vi "from string.vi"(8 "error in":errorcluster, 9 "data":string, 10 "version":string, 11 "CEF_Configuration in":refnum<class "XY Plotter configuration.lvclass">) -> (0 "error out":errorcluster, 3 "CEF_Configuration out":refnum<class "XY Plotter configuration.lvclass">)   [LabVIEW 2025, in "XY Plotter.lvlib" / "XY Plotter configuration.lvclass"]
doc: "Provides an interface for loading a module configuration from a file or other serialized data source. It is recommended that all children of this class store data in two sets--data required for its own initialization, and any data required for parent initialization--and that each implementation uses the <b>Call Parent Method</b> primitive to de-serialize parent information.Copyright 2017 National Instruments Corporation\n\nLicensed under the Apache License, Version 2.0 (the \"License\"); you may not use this file except in compliance with the License. You may obtain a copy of the License at http://www.apache.org/licenses/LICENSE-2.0\nUnless required by applicable law or agreed to in writing, software distributed under the License is distributed on an \"AS IS\" BASIS, WITHOUT WARRANTIES OR CONDITIONS OF ANY KIND, either express or implied. See the License for the specific language governing permissions and limitations under the License."
uses:
  XY Plotter configuration.lvclass
  XY Plotter.ctl
  XY Plotter configuration.lvclass/XY Plotter configuration.ctl
  4cdf8148-81d7-474d-a8fa-f40dbeba2f75.vi
  <vilib>/JDP Science/JSONtext/JSON text to Variant.vi
  <vilib>/JDP Science/JSONtext/LVClass Serializer/JSONtext LVClass Serializer.lvclass
  Users/Public/Documents/Sandia National Labs/TSS Plugin/CEF.lvlibp/serializable configuration/CEF_serializable configuration.lvclass
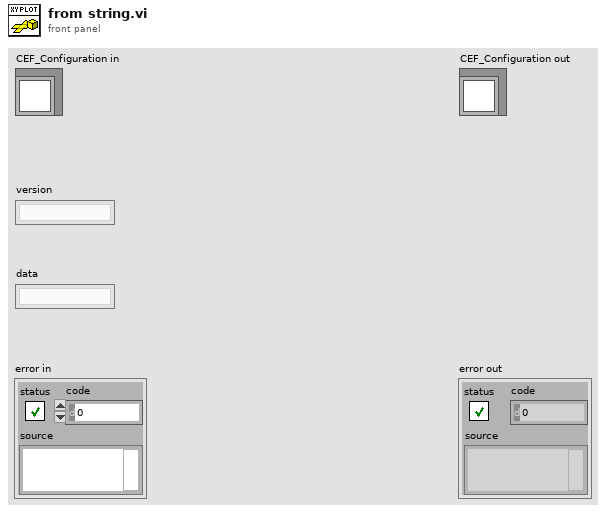
[diagram p1: front panel]
types:
  T1 = typedef "XY Plotter.lvlib/XY Plotter configuration.lvclass/XY Plotter.ctl" = cluster{"Data Rate":i32, "Y-Scales":cluster{"Label":string, "Max":dbl, "Min":dbl, "Unit":enum16{"---", "V", "mA", "sec", "dB", "deg", "in/s", "in", "lbf", "Hz", "psi", "gpm"}, "Visible":bool}[], "Note":string, "History Length":i32, "DataLog Path":path, "Plot type":bool, "X-Scales":cluster{"Label":string, "Max":dbl, "Min":dbl, "Unit":enum16{"---", "V", "mA", "sec", "dB", "deg", "in/s", "in", "lbf", "Hz", "psi", "gpm"}, "Visible":bool}[], "Plot List":cluster{"Plot Name":string, "X Scale Index":u32, "Y Scale Index":u32, "Visible":bool}[]}
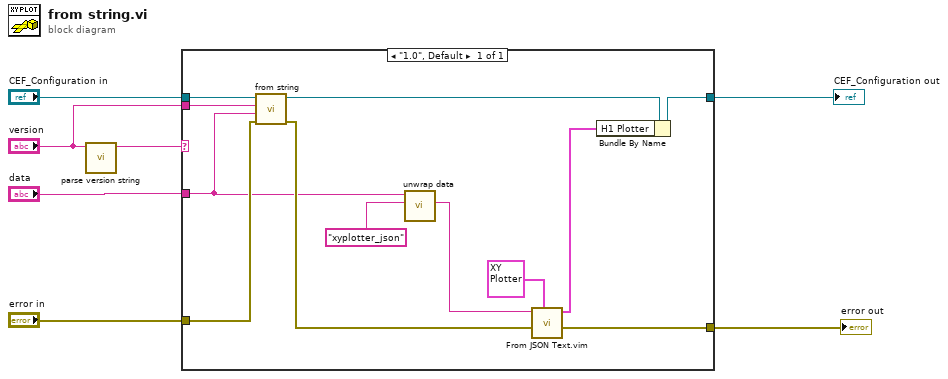
[diagram p0: block diagram]
diagram:
  n1 = call "parse version string.vi"("full version"="version") -> ("major.minor version"=w7:string)  [unwired: 7 in, 3 out]
  n2 = case shown="\"1.0\", Default" w7 {
    tunnel: "CEF_Configuration in" -> [w19]
    tunnel: [w15] -> w4
    tunnel: "data" -> [w11]
    tunnel: "error in" -> [w17]
    tunnel: [w10] -> w5
    tunnel: "version" -> [w12]
    frame "1.0", Default {
      n3 = call-parent "from string.vi"("error in"=w17, "data"=w11, "version"=w12, "CEF_Configuration in"=w19) -> ("error out"=w16:errorcluster, "CEF_Configuration out"=w18:refnum<class "XY Plotter configuration.lvclass">)  [unwired: 6 in]
      n4 = call "unwrap data.vi"("identifier"="xyplotter_json" ("additional identifier"), "data to unwrap"=w11) -> ("unwrapped data"=w13:string)  [unwired: 8 in, 1 out]
      n5 = call "From JSON Text.vim"("Data Type and Default Value"=T1 {"Data Rate"=20, "Y-Scales"=[{"Label"="Amplitude", "Max"=5.0, "Min"=-5.0, "Unit"=enum."in", "Visible"=TRUE}, {"Label"="", "Max"=100.0, "Min"=-100.0, "Unit"=enum."---", "Visible"=TRUE}], "Note"="", "History Length"=5, "DataLog Path"=path "C:/_Data_Log", "Plot type"=FALSE, "X-Scales"=[{"Label"="Amplitude", "Max"=5.0, "Min"=-5.0, "Unit"=enum."in", "Visible"=TRUE}, {"Label"="", "Max"=100.0, "Min"=-100.0, "Unit"=enum."---", "Visible"=TRUE}], "Plot List"=[{"Plot Name"="Ch1", "X Scale Index"=0, "Y Scale Index"=0, "Visible"=TRUE}, {"Plot Name"="Ch1", "X Scale Index"=0, "Y Scale Index"=0, "Visible"=TRUE}]} ("H1 Plotter Setting"), "error in (no error)"=w16, "JSON"=w13) -> ("error out"=w10:errorcluster, "Data out"=w9:T1)  [unwired: 7 in]
      n6 = Bundle By Name(cluster=w18, "H1 Plotter"=w9) -> (w15:refnum<class "XY Plotter configuration.lvclass">)
    }
  }
  "error out" <- w5
  "CEF_Configuration out" <- w4
